vi "06c-arrays.vi"() -> ()   [LabVIEW 2018, in "LV2Julia_examples.lvlib"]
uses:
  LV2Julia_examples.lvlib
  LV2Julia_core/VIs/Server or client state.ctl
  statistics.ctl
  LV2Julia_core/VIs/Commands.ctl
  LV2Julia_core/VIs/ZMQ timeouts.ctl
  0d29fc62-3d1d-4713-a954-9c9e873b3633.vi
  aea790a6-a42b-4eb0-905f-734239196901.vi
  72a46192-383e-4ee5-9465-71670922b82a.vi
  ef5408d4-6538-41d1-b296-fda05a71e4b0.vi
  b8d67b76-17b0-4ad8-b521-2f6549c52c10.vi
  e4efb182-1b04-4d49-96a3-1defebd055ea.vi
  ef458cb0-9ca2-4aa9-bd1e-ad103f8bb0c0.vi
  9df197b6-2616-4b86-abf4-a70e9215d122.vi
  28751878-cf8c-4743-a8b0-c60d78ce5b36.vi
  c328879f-33e1-4261-a6aa-c93c9ebac265.vi
  0d29fc62-3d1d-4713-a954-9c9e873b3633.vi/8ee49078-a04b-40cf-aceb-de90d52f19ef.vi
  aea790a6-a42b-4eb0-905f-734239196901.vi/353007a7-a356-474a-8eac-0d4386ef6058.vi
  72a46192-383e-4ee5-9465-71670922b82a.vi/c983efa1-af68-42af-ad76-fb72a003131c.vi
  ef5408d4-6538-41d1-b296-fda05a71e4b0.vi/79acbf14-e29b-47e7-ab31-61d634111b06.vi
  b8d67b76-17b0-4ad8-b521-2f6549c52c10.vi/ce4ba451-f191-4dd3-bdbe-afda97c3e90b.vi
  e4efb182-1b04-4d49-96a3-1defebd055ea.vi/38283ee9-2e49-4cb4-9e09-483ddbb25034.vi
  e4efb182-1b04-4d49-96a3-1defebd055ea.vi/77e4dc6e-2a6f-4cba-b1e6-347186ad7875.vi
  e4efb182-1b04-4d49-96a3-1defebd055ea.vi/b97adf4a-ed5a-4736-8d10-e745d89490c3.vi
  e4efb182-1b04-4d49-96a3-1defebd055ea.vi/d0fc0203-bfc6-4e6c-8f24-5bc77162b354.vi
  ef458cb0-9ca2-4aa9-bd1e-ad103f8bb0c0.vi/e8b90c0a-49a5-4093-b01b-c91da666bc06.vi
  9df197b6-2616-4b86-abf4-a70e9215d122.vi/e9d8b799-20ce-4ea8-8afd-a7c3f5f9bac5.vi
  28751878-cf8c-4743-a8b0-c60d78ce5b36.vi/d1f7fe03-3423-447d-95f9-53f6532833c0.vi
  c328879f-33e1-4261-a6aa-c93c9ebac265.vi/c8923e2a-1ded-4353-bc92-8b7bded5bb04.vi
  c328879f-33e1-4261-a6aa-c93c9ebac265.vi/96e499ba-e0b1-454e-8d08-26b47ac44832.vi
  c328879f-33e1-4261-a6aa-c93c9ebac265.vi/4642b7d4-ce05-4ce2-a42b-a73aa147d3f7.vi
  c328879f-33e1-4261-a6aa-c93c9ebac265.vi/f9786830-7ae8-42d9-8a4c-51c42e73d889.vi
  72a46192-383e-4ee5-9465-71670922b82a.vi/c983efa1-af68-42af-ad76-fb72a003131c.vi/33b6bc94-2c06-4568-8114-f216ba0f03de.vi
  ef5408d4-6538-41d1-b296-fda05a71e4b0.vi/79acbf14-e29b-47e7-ab31-61d634111b06.vi/cc2bbb06-afa0-4be4-919e-a8fae2c74d3e.vi
  b8d67b76-17b0-4ad8-b521-2f6549c52c10.vi/ce4ba451-f191-4dd3-bdbe-afda97c3e90b.vi/d6ff21e3-b3c7-4fa3-9ab2-84006c57fe85.vi
  b8d67b76-17b0-4ad8-b521-2f6549c52c10.vi/ce4ba451-f191-4dd3-bdbe-afda97c3e90b.vi/08390940-31fa-46fd-b0fe-c03a9e9ae5e0.vi
  b8d67b76-17b0-4ad8-b521-2f6549c52c10.vi/ce4ba451-f191-4dd3-bdbe-afda97c3e90b.vi/f2515907-fae4-4c80-a8e6-e5824cff5167.vi
  e4efb182-1b04-4d49-96a3-1defebd055ea.vi/38283ee9-2e49-4cb4-9e09-483ddbb25034.vi/ce185c6b-02c1-4169-bc67-9a48479340ad.vi
  e4efb182-1b04-4d49-96a3-1defebd055ea.vi/38283ee9-2e49-4cb4-9e09-483ddbb25034.vi/fde1154f-94cd-44ba-b83c-2af9a583bb9b.vi
  9df197b6-2616-4b86-abf4-a70e9215d122.vi/e9d8b799-20ce-4ea8-8afd-a7c3f5f9bac5.vi/5df9f504-bb34-4e76-bc55-8e28577d31a1.vi
  28751878-cf8c-4743-a8b0-c60d78ce5b36.vi/d1f7fe03-3423-447d-95f9-53f6532833c0.vi/e8edbf9e-669d-446f-81ac-d0e3a30402fa.vi
  28751878-cf8c-4743-a8b0-c60d78ce5b36.vi/d1f7fe03-3423-447d-95f9-53f6532833c0.vi/defc33f1-9e74-4a4a-aa1e-fd177d6d2623.vi
  28751878-cf8c-4743-a8b0-c60d78ce5b36.vi/d1f7fe03-3423-447d-95f9-53f6532833c0.vi/5cacfdae-5585-4b52-a326-4693d1b4fdf6.vi
  c328879f-33e1-4261-a6aa-c93c9ebac265.vi/c8923e2a-1ded-4353-bc92-8b7bded5bb04.vi/c265a51a-1fb2-4459-9c45-821212f90ae1.vi
  c328879f-33e1-4261-a6aa-c93c9ebac265.vi/c8923e2a-1ded-4353-bc92-8b7bded5bb04.vi/92df87ef-9624-4d14-9ddb-e8648c3f0517.vi
  72a46192-383e-4ee5-9465-71670922b82a.vi/c983efa1-af68-42af-ad76-fb72a003131c.vi/33b6bc94-2c06-4568-8114-f216ba0f03de.vi/f9ef1e04-5461-4325-a87b-15ec0fff3bc2.vi
  ef5408d4-6538-41d1-b296-fda05a71e4b0.vi/79acbf14-e29b-47e7-ab31-61d634111b06.vi/cc2bbb06-afa0-4be4-919e-a8fae2c74d3e.vi/de5872c4-2e9b-436f-ba6d-4399df224a15.vi
  e4efb182-1b04-4d49-96a3-1defebd055ea.vi/38283ee9-2e49-4cb4-9e09-483ddbb25034.vi/ce185c6b-02c1-4169-bc67-9a48479340ad.vi/a8ea3af6-7f77-41b1-ad32-9e59f4b2dbd8.vi
  9df197b6-2616-4b86-abf4-a70e9215d122.vi/e9d8b799-20ce-4ea8-8afd-a7c3f5f9bac5.vi/5df9f504-bb34-4e76-bc55-8e28577d31a1.vi/71f381b8-1ffb-4949-90c1-ed40c9115f9c.vi
  c328879f-33e1-4261-a6aa-c93c9ebac265.vi/c8923e2a-1ded-4353-bc92-8b7bded5bb04.vi/c265a51a-1fb2-4459-9c45-821212f90ae1.vi/d2714d2a-197e-4f23-9508-d3947c608829.vi
  LV2Julia_core/VIs/check ID validity.vi
  LV2Julia_core/VIs/bindata_descr to JSON.vi
  LV2Julia_core/VIs/check cluster field names.vi
  LV2Julia_core/VIs/concat JSON.vi
  LV2Julia_core/VIs/build request.vi
  LV2Julia_core/VIs/Parse server response.vi
  LV2Julia_core/VIs/log jl exceptions.vi
  <vilib>/Utility/error.llb/Error Cluster From Error Code.vi
  LV2Julia_core/LV2Julia_core.lvlib
panel:
  out "Statistics 1":T1={"size "=0, "mean"=nan, "median"=nan, "min"=nan, "max"=nan} caption="Statistics (ms)" {"min" format="%#.1f"; "max" format="%#.1f"; "median" format="%.1f"; "mean" format="%.1f"}
  in  "max size 1":i32=20 caption="sample max"
  out "Statistics 2":T1={"size "=0, "mean"=nan, "median"=nan, "min"=nan, "max"=nan} caption="Statistics (ms)" {"min" format="%#.1f"; "max" format="%#.1f"; "median" format="%.1f"; "mean" format="%.1f"}
  in  "max size 2":i32=20 caption="sample max"
  out "error info 2":string
  out "call duration (ms) 2":dbl format="%#.3f"
  in  "N - arr size 2":u16=4
  out "Input Matrix (NxN)2":dbl[][](array[numeric])=[[1.0, 0.0, 5.0], [4.0, 2.0, 1.0], [2.0, 2.0, 3.0]] format="%#.4g"
  in  "paus2":bool
  out "current error 2":errorcluster
  out "error info 1":string
  out "call duration (ms) 1":dbl format="%#.3f"
  in  "N - arr size 1":u16=4
  out "Solution Vector":dbl[](array[numeric]) format="%.4f"
  out "Known Vector":dbl[](array[numeric])=[22.0, 14.0, 18.0] format="%#.4g"
  out "Input Matrix (NxN) 1":dbl[][](array[numeric])=[[1.0, 0.0, 5.0], [4.0, 2.0, 1.0], [2.0, 2.0, 3.0]] format="%#.4g"
  in  "paus1":bool
  out "current error 1":errorcluster
  out "Eigenvalues":cdb[](array[numeric]) format="%.2f"
  out "final error":errorcluster
  in  "stop":bool
  out "ZMQ timeout":bool
  out "Jl Server state":T2
  # "Concurrent access to Julia server: Solving a system of linear equations in one loop, and computing eigenvalues in another one."
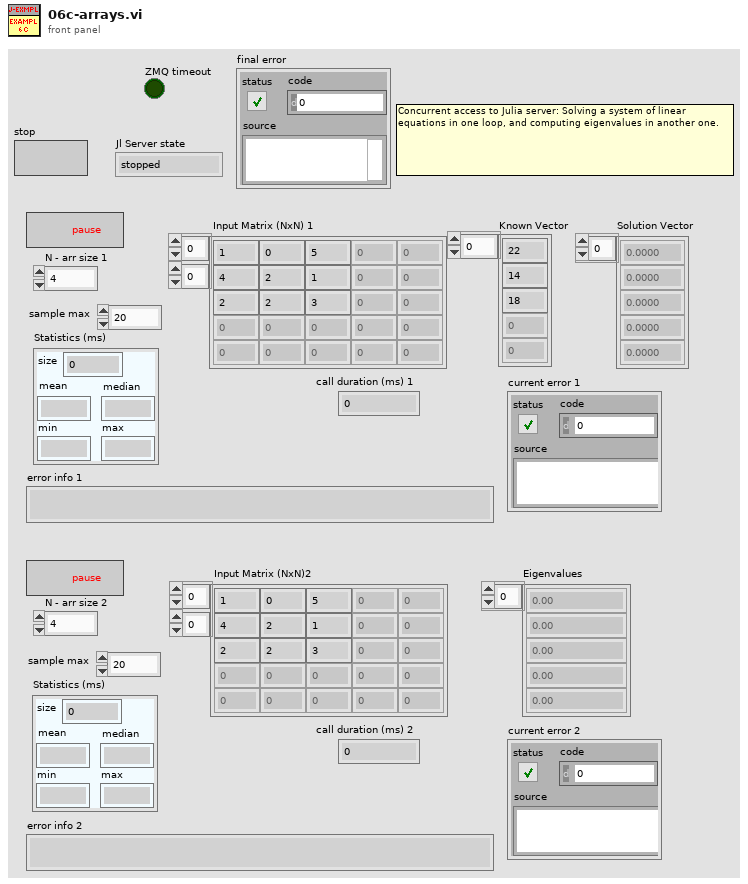
[diagram p1: front panel]
types:
  T1 = typedef "LV2Julia_examples.lvlib/statistics.ctl" = cluster{"size ":u32, "mean":dbl, "median":dbl, "min":dbl, "max":dbl}
  T2 = typedef "LV2Julia_core.lvlib/Server or client state.ctl" = enum16{"stopped", "running", "unknown"}
  T3 = typedef "LV2Julia_core.lvlib/ZMQ timeouts.ctl" = cluster{"SNDTIMEO":i32, "RCVTIMEO":i32}
  T4 = typedef "LV2Julia_core.lvlib/Commands.ctl" = enum16{"Start Jl-server & Init LV-client", "Send request & Get response ", "Stop Jl-server & Cleanup LV-client", "Cleanup LV-client", "Start Jl-server", "Stop Jl-server", "Init LV-Client", "Cleanup LV-Client", "(not allowed)", "Set LV Client state", "Set Jl Server state", "set ZMQ timeout", "read ZMQ timeout", "read-out state"}
  T5 = typedef "LV2Julia_core.lvlib/Bindata&description.ctl" = cluster{"bindata_descr":T6[], "bindata":u8[]}
  T6 = typedef "LV2Julia_core.lvlib/Bindata description.ctl" = cluster{"nofbytes":i32, "numtype":string, "start":i32, "arrdims":i32[], "kwarg_name":string, "category":string}
  T7 = typedef "LV2Julia_core.lvlib/detailed error info.ctl" = cluster{"exception_or_info":string, "trace":T8[]}
  T8 = typedef "LV2Julia_core.lvlib/StackFrame.ctl" = cluster{"frame_summary":string, "func":string, "linfo":string, "file":string, "line":i32, "pointer":u64, "from_c":bool, "inlined":bool}
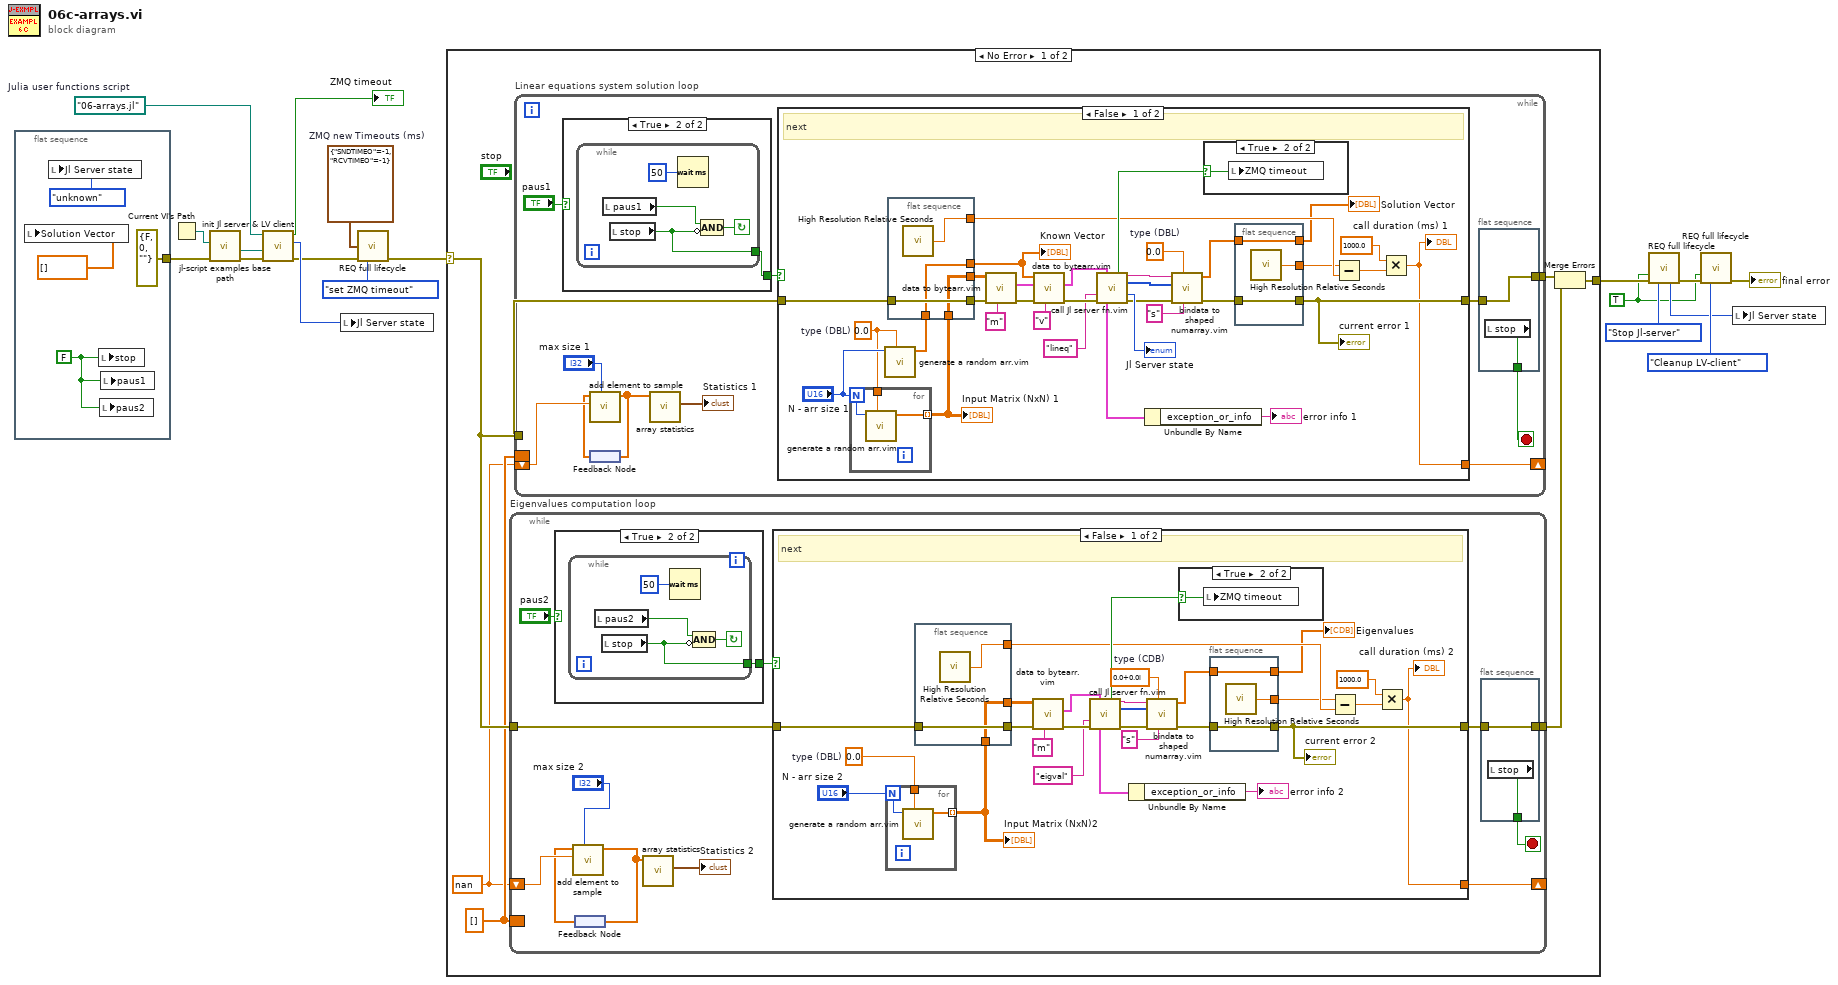
[diagram p0: block diagram]
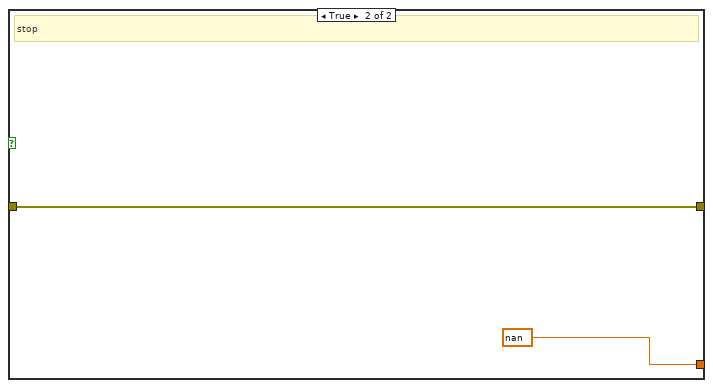
[diagram p4: hidden frame]
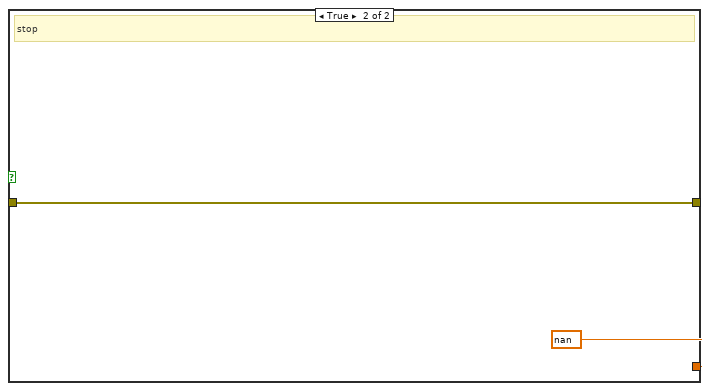
[diagram p7: hidden frame]
diagram:
  w9 = T3 {"SNDTIMEO"=-1, "RCVTIMEO"=-1}  # ZMQ new Timeouts (ms)
  w8 = path "06-arrays.jl"  # Julia user functions script
  w12 = TRUE ("Force command")
  n1 = flat-sequence {
    tunnel: [errorcluster {"status"=FALSE, "code"=0, "source"=""} ("error in (no error)")] -> w1
    frame #0 {
      w19 = FALSE ("stop")
      n2 = local write "Solution Vector"(dbl[] [] ("Server response")) -> ()
      n3 = local write "Jl Server state"(Server_or_client_state."unknown" ("Jl Server state out")) -> ()
      n4 = local write "stop"(w19) -> ()
      n5 = local write "paus2"(w19) -> ()
      n6 = local write "paus1"(w19) -> ()
    }
  }
  n7 = Current VI's Path() -> (path=w4:path)
  n8 = call "jl-script examples base path.vi"("error in (no error)"=w1, "calling example VI path"=w4) -> ("error out"=w3:errorcluster, "jl-script-examples base path"=w2:path)  [unwired: 8 in]
  n9 = call "init Jl server & LV client.vi"("error in (no error)"=w3, "Base path (not a path)"=w2, "Julia user functions script"=w8) -> ("error out"=w5:errorcluster, "Jl Server state out"=w6:T2, "timeout?"=→"ZMQ timeout":bool)  [unwired: 3 in, 3 out]
  n10 = local write "Jl Server state"(w6) -> ()
  n11 = call "REQ full lifecycle.vi"("ZMQ new Timeouts in"=w9, "error in"=w5, "command"=Commands."set ZMQ timeout") -> ("error out"=w11:errorcluster)  [unwired: 6 in, 6 out]
  n12 = case shown="No Error" w11 {
    selector: w11 -> [w25 w152]
    tunnel: [w27 w152] -> w18
    frame No Error {
      w24 = dbl[] []
      w23 = nan
      n13 = while "Eigenvalues computation loop" {
        tunnel: w25 -> [w40]
        tunnel: [w38] -> w26
        shift-right: [w34] -> _
        shift-left: w23 -> [w33]
        border: w24 -> [_]
        stop <- w37 stop-if-true
        n14 = case shown="True" "paus2" {
          tunnel: [_ w41] -> w36
          frame False {
          }
          frame True {
            n15 = while {
              tunnel: [w42] -> w41
              stop <- w43 continue-if-true
              n16 = local read "paus2"() -> (w44:bool)
              n17 = local read "stop"() -> (w42:bool)
              n18 = Wait (ms)(milliseconds to wait=u32 50) -> ()  [unwired: 1 out]
              n19 = Compound Arithmetic op=AND(w44, invert w42) -> (w43:bool)
            }
          }
        }
        n20 = feedback #1() -> (w30:dbl[])
        n21 = call "add element to sample.vi"("sample size in"="max size 2", "element in"=w33, "Array in"=w30) -> ("Array out"=w32:dbl[])  [unwired: 8 in]
        n22 = feedback-in #1(w32) -> ()
        n23 = call "array statistics.vi"("Array in"=w32) -> ("Statistics (ms)"=→"Statistics 2":T1)  [unwired: 10 in]
        n24 = case shown="False" w36 {
          tunnel: [w53 w86] -> w39
          tunnel: w40 -> [w64 w86]
          tunnel: [w50 nan] -> w34
          frame False {
            w71 = 0.0  # type (DBL)
            w73 = cdb 0.0+0.0i  # type (CDB)
            # "next"
            n25 = for {
              N: "N - arr size 2" -> [w81]
              tunnel: [w83] -> w54 mode=indexing
              tunnel: w71 -> [w82]
              n26 = call "generate a random arr.vim"("type in"=w82, "arr size"=w81) -> ("float out"=w83:dbl[])  [unwired: 5 in, 4 out]
            }
            "Input Matrix (NxN)2" <- w54
            n27 = flat-sequence {
              tunnel: [w80] -> w63
              tunnel: w64 -> [w80]
              tunnel: w54 -> [w79]
              tunnel: [w79] -> w62
              tunnel: [w78] -> w60
              frame #0 {
                n28 = call <vilib>:"High Resolution Relative Seconds.vi"() -> ("relative seconds"=w78:dbl)
              }
            }
            n29 = call "data to bytearr.vim"("kwarg_name"="m", "error in (no error)"=w63, "data in"=w62) -> ("error out"=w65:errorcluster, "Bindata & descr out"=w69:T5)  [unwired: 6 in, 1 out]
            n30 = call "call Jl server fn.vim"("Bindata & descr in"=w69, "fun2call"="eigval" ("Julia function name"), "error in (no error)"=w65) -> ("timeout?"=w68:bool, "JSON received"=w67:string, "binary data received"=w66:u8[], "detailed error info"=w55:T7, "error out"=w70:errorcluster)  [unwired: 6 in, 2 out]
            n31 = Unbundle By Name(w55) -> ("exception_or_info"=→"error info 2":string)
            n32 = call "bindata to shaped numarray.vim"("name"="s" ("kwarg_name"), "element type"=w73, "error in (no error)"=w70, "binary data"=w66, "JSON in"=w67) -> ("error out"=w61:errorcluster, "numarray 1D"=w49:cdb[])  [unwired: 1 in, 4 out]
            n33 = case shown="True" w68 {
              selector: w68 -> [_ w84]
              frame False {
              }
              frame True {
                n34 = local write "ZMQ timeout"(w84) -> ()
              }
            }
            n35 = flat-sequence {
              tunnel: [w77] -> w53
              tunnel: w61 -> [w77]
              tunnel: [w76] -> w57
              tunnel: [w75] -> w48
              tunnel: w49 -> [w75]
              frame #0 {
                n36 = call <vilib>:"High Resolution Relative Seconds.vi"() -> ("relative seconds"=w76:dbl)
              }
            }
            n37 = Subtract(x=w57, y=w60) -> (x-y=w59:dbl)
            n38 = Multiply(x=1000.0, y=w59) -> (x*y=w50:dbl)
            "call duration (ms) 2" <- w50
            "Eigenvalues" <- w48
            "current error 2" <- w53
          }
          frame True {
            # "stop"
          }
        }
        n39 = flat-sequence {
          tunnel: w39 -> [w47]
          tunnel: [w47] -> w38
          tunnel: [w46] -> w37
          frame #0 {
            n40 = local read "stop"() -> (w46:bool)
          }
        }
      }
      n41 = while "Linear equations system solution loop" {
        tunnel: w25 -> [w93]
        tunnel: [w97] -> w28
        shift-right: [w92] -> _
        shift-left: w23 -> [w91]
        border: w24 -> [_]
        stop <- w96 stop-if-true
        n42 = case shown="True" "paus1" {
          tunnel: [_ w99] -> w95
          frame False {
          }
          frame True {
            n43 = while {
              tunnel: [w100] -> w99
              stop <- w101 continue-if-true
              n44 = local read "paus1"() -> (w102:bool)
              n45 = local read "stop"() -> (w100:bool)
              n46 = Wait (ms)(milliseconds to wait=u32 50) -> ()  [unwired: 1 out]
              n47 = Compound Arithmetic op=AND(w102, invert w100) -> (w101:bool)
            }
          }
        }
        n48 = feedback #2() -> (w89:dbl[])
        n49 = call "add element to sample.vi"("sample size in"="max size 1", "element in"=w91, "Array in"=w89) -> ("Array out"=w90:dbl[])  [unwired: 8 in]
        n50 = feedback-in #2(w90) -> ()
        n51 = call "array statistics.vi"("Array in"=w90) -> ("Statistics (ms)"=→"Statistics 1":T1)  [unwired: 10 in]
        n52 = case shown="False" w95 {
          tunnel: [w109 w151] -> w98
          tunnel: w93 -> [w124 w151]
          tunnel: [w108 nan] -> w92
          frame False {
            w132 = 0.0  # type (DBL)
            w135 = 0.0  # type (DBL)
            # "next"
            n53 = for {
              N: "N - arr size 1" -> [w146]
              tunnel: [w148] -> w116 mode=indexing
              tunnel: w132 -> [w147]
              n54 = call "generate a random arr.vim"("type in"=w147, "arr size"=w146) -> ("float out"=w148:dbl[])  [unwired: 5 in, 4 out]
            }
            "Input Matrix (NxN) 1" <- w116
            n55 = call "generate a random arr.vim"("type in"=w132, "arr size"="N - arr size 1") -> ("float out"=w121:dbl[])  [unwired: 5 in, 4 out]
            n56 = flat-sequence {
              tunnel: [w145] -> w123
              tunnel: w124 -> [w145]
              tunnel: w116 -> [w144]
              tunnel: [w144] -> w122
              tunnel: [w143] -> w111
              tunnel: w121 -> [w143]
              tunnel: [w142] -> w119
              frame #0 {
                n57 = call <vilib>:"High Resolution Relative Seconds.vi"() -> ("relative seconds"=w142:dbl)
              }
            }
            n58 = call "data to bytearr.vim"("kwarg_name"="m", "error in (no error)"=w123, "data in"=w122) -> ("error out"=w138:errorcluster, "Bindata & descr out"=w137:T5)  [unwired: 6 in, 1 out]
            n59 = call "data to bytearr.vim"("kwarg_name"="v", "error in (no error)"=w138, "Bindata & descr in"=w137, "data in"=w111) -> ("error out"=w125:errorcluster, "Bindata & descr out"=w129:T5)  [unwired: 5 in, 1 out]
            n60 = call "call Jl server fn.vim"("Bindata & descr in"=w129, "fun2call"="lineq" ("Julia function name"), "error in (no error)"=w125) -> ("timeout?"=w128:bool, "JSON received"=w127:string, "binary data received"=w126:u8[], "Jl Server state out"=→"Jl Server state":T2, "detailed error info"=w113:T7, "error out"=w130:errorcluster)  [unwired: 6 in, 1 out]
            n61 = Unbundle By Name(w113) -> ("exception_or_info"=→"error info 1":string)
            n62 = call "bindata to shaped numarray.vim"("name"="s" ("kwarg_name"), "element type"=w135, "error in (no error)"=w130, "binary data"=w126, "JSON in"=w127) -> ("error out"=w120:errorcluster, "numarray 1D"=w107:dbl[])  [unwired: 1 in, 4 out]
            n63 = case shown="True" w128 {
              selector: w128 -> [_ w149]
              frame False {
              }
              frame True {
                n64 = local write "ZMQ timeout"(w149) -> ()
              }
            }
            n65 = flat-sequence {
              tunnel: [w141] -> w109
              tunnel: w120 -> [w141]
              tunnel: [w140] -> w115
              tunnel: [w139] -> w106
              tunnel: w107 -> [w139]
              frame #0 {
                n66 = call <vilib>:"High Resolution Relative Seconds.vi"() -> ("relative seconds"=w140:dbl)
              }
            }
            n67 = Subtract(x=w115, y=w119) -> (x-y=w118:dbl)
            n68 = Multiply(x=1000.0, y=w118) -> (x*y=w108:dbl)
            "call duration (ms) 1" <- w108
            "current error 1" <- w109
            "Known Vector" <- w111
            "Solution Vector" <- w106
          }
          frame True {
            # "stop"
          }
        }
        n69 = flat-sequence {
          tunnel: w98 -> [w105]
          tunnel: [w105] -> w97
          tunnel: [w104] -> w96
          frame #0 {
            n70 = local read "stop"() -> (w104:bool)
          }
        }
      }
      n71 = Merge Errors(w28, w26) -> (w27:errorcluster)
    }
    frame Error {
    }
  }
  n72 = call "REQ full lifecycle.vi"("Force command"=w12, "error in"=w18, "command"=Commands."Stop Jl-server") -> ("Jl Server state out"=w13:T2, "error out"=w16:errorcluster)  [unwired: 6 in, 5 out]
  n73 = call "REQ full lifecycle.vi"("Force command"=w12, "error in"=w16, "command"=Commands."Cleanup LV-client") -> ("error out"=→"final error":errorcluster)  [unwired: 6 in, 6 out]
  n74 = local write "Jl Server state"(w13) -> ()
